vi "FuncVI-NotifDestroy.vi"(5 "InstanceRef":T2, 9 "arg list":T1[](array[typedef]) {"num" format="%.2f"}) -> (0 "error out":bool, 3 "result":T1 {"num" format="%.2f"})   [LabVIEW 2021]
doc: "::: CalcExpress Toolkit :::\nCopyright (c) 2000-2026 Konstantin Shifershteyn. All rights reserved."
uses:
  cetypes.llb/CalcExpress Function Argument Info.ctl
  cetypes.llb/CalcExpress Instance RefNum.ctl
panel:
  in  "max arg num":i32=1
  in  "min arg num":i32=1
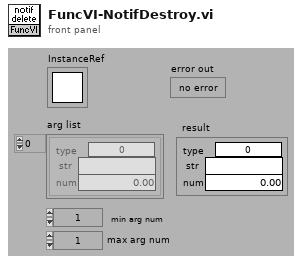
[diagram p1: front panel]
types:
  T1 = typedef "CalcExpress Function Argument Info.ctl" = cluster{"type":u32, "str":string, "num":dbl}
  T2 = typedef "CalcExpress Instance RefNum.ctl" = refnum<k1>
  T3 = enum32{"String", "DBL Number", "identifier", "1D Array of DBL", "2D Array of DBL", "CDB Number", "1D Array of CDB", "2D Array of CDB", "1D Array of String", "2D Array of String", "Unknown data type"}
  T4 = cluster{"data type":enum32{"String", "DBL Number", "identifier", "1D Array of DBL", "2D Array of DBL", "CDB Number", "1D Array of CDB", "2D Array of CDB", "1D Array of String", "2D Array of String", "Unknown data type"}, "str":string, dbl}
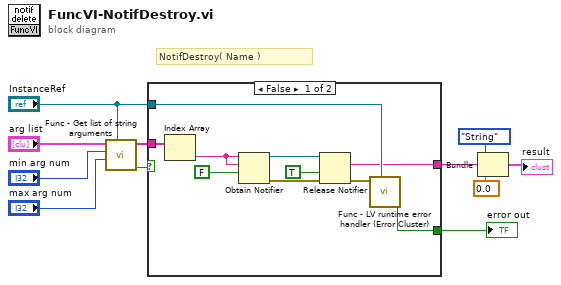
[diagram p0: block diagram]
diagram:
  # "NotifDestroy( Name )"
  n1 = call "Func - Get list of string arguments.vi"("InstanceRef"="InstanceRef", "max arg num"="max arg num", "min arg num"="min arg num", "arg list"="arg list") -> ("error out"=w4:bool, "val list"=w10:string[])  [unwired: 4 in]
  n2 = case shown="False" w4 {
    selector: w4 -> [_ w22]
    tunnel: w10 -> [w21 _]
    tunnel: [w14 _] -> w6
    tunnel: "InstanceRef" -> [w20 _]
    tunnel: [w19 w22] -> w3
    frame False {
      n3 = Index Array(array=w21) -> (element=w12:string)  [unwired: 1 in]
      n4 = Obtain Notifier(name (unnamed)=w12, notification data type=w12, create if not found? (T)=FALSE) -> (notifier out=w15:refnum<notifier>, error out=w18:errorcluster)  [unwired: 1 in, 1 out]
      n5 = Release Notifier(notifier=w15, force destroy? (F)=TRUE, error in (no error)=w18) -> (last notification=w14:string, error out=w13:errorcluster)  [unwired: 1 out]
      n6 = call "Func - LV runtime error handler (Error Cluster).vi"("InstanceRef"=w20, "LabVIEW error"=w13) -> ("error out"=w19:bool)  [unwired: 4 in, 3 out]
    }
    frame True {
    }
  }
  "error out" <- w3
  n7 = Bundle("data type"=T3."String", "str"=w6, 0.0) -> (→"result":T4)  [unwired: 1 in]
